vi "ex3.vi"() -> ()   [LabVIEW 2025]
panel:
  out "Numeric":i32
  in  "D":u32 format="%b"
  out "CRC 2":u32 format="%b"
  out "Message with CRC 2":u32 format="%b"
  out "Message":u32 format="%b"
  out "CRC":u32 format="%b"
  in  "Message with CRC":u32 format="%b"
  # "Decoder"
  # "Enkoder"
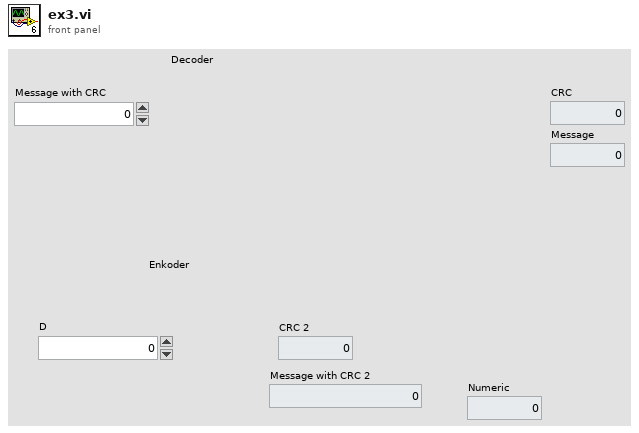
[diagram p1: front panel]
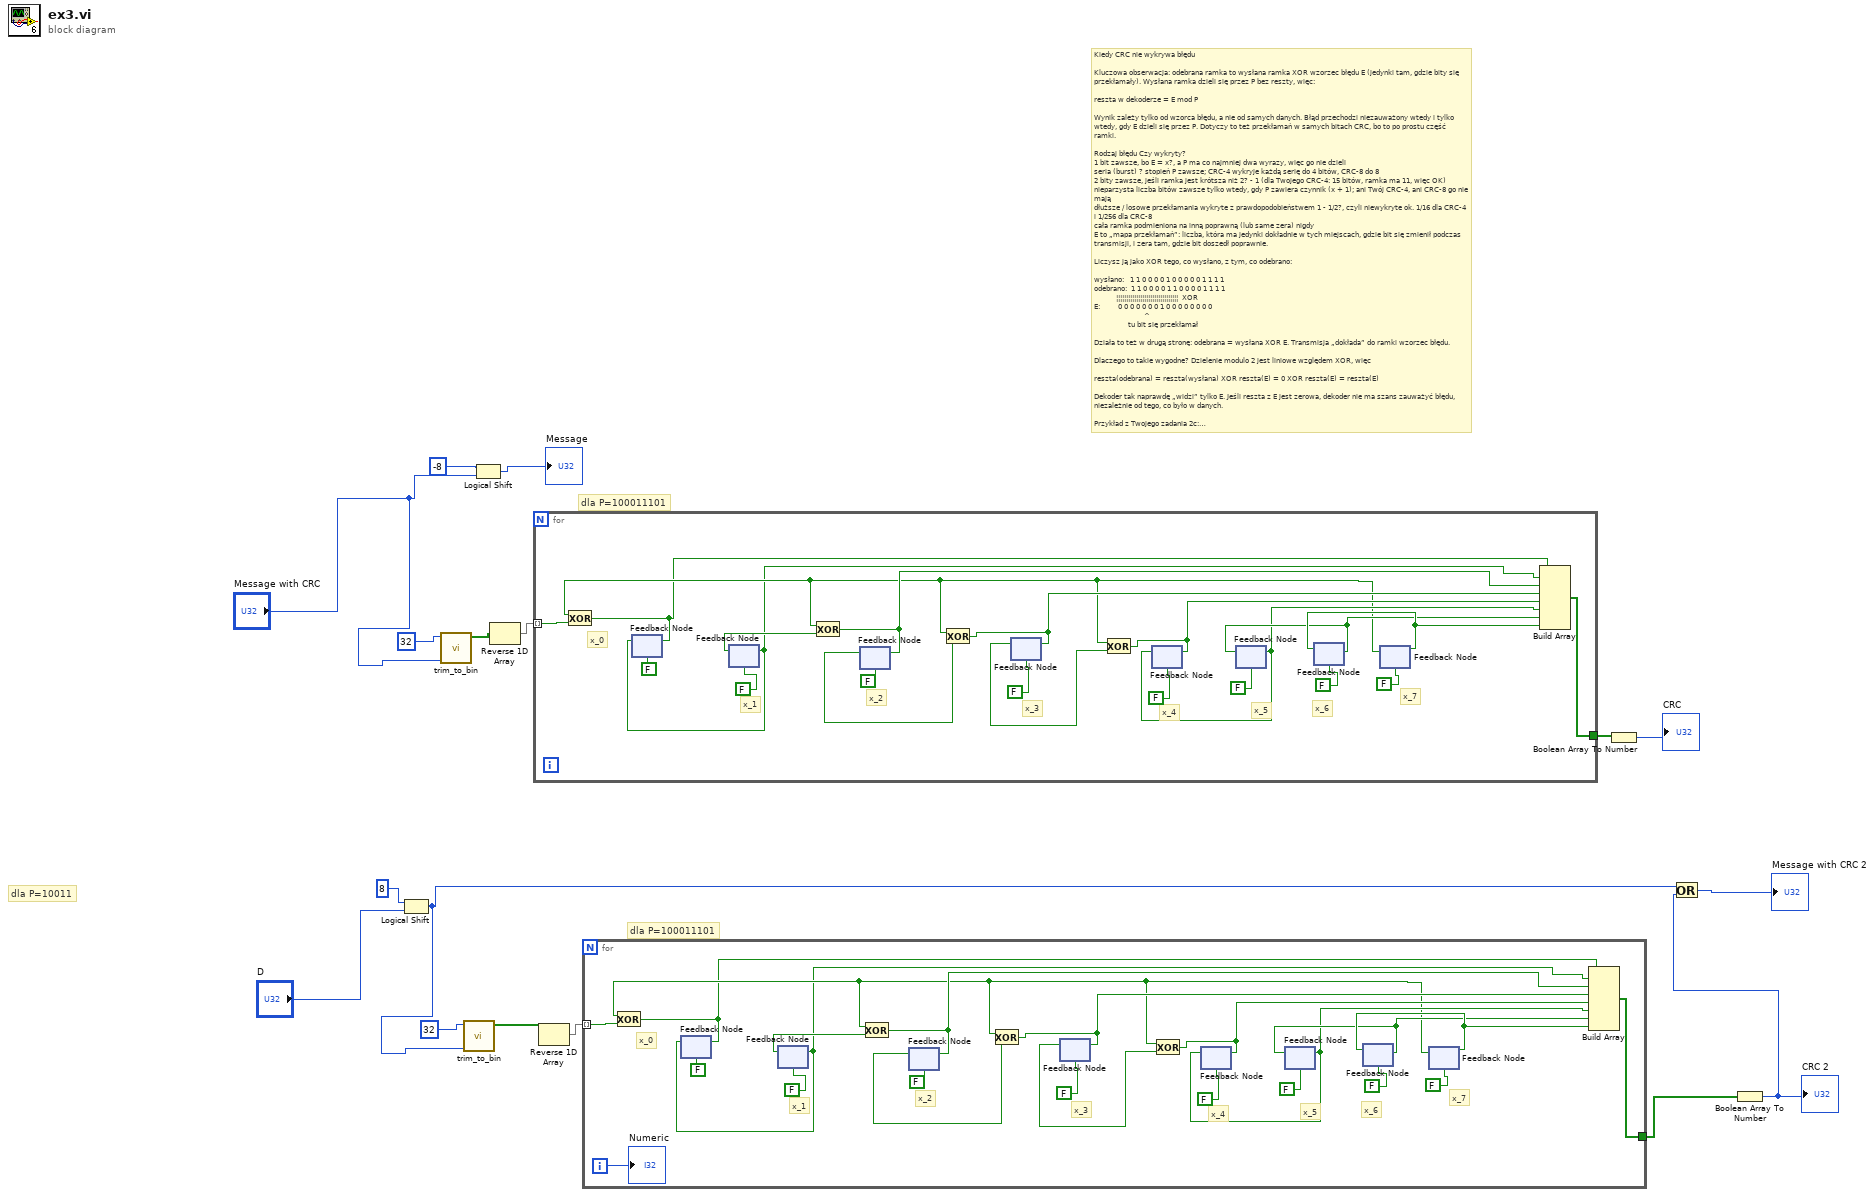
[diagram p0: block diagram]
diagram:
  # "Kiedy CRC nie wykrywa błędu\n\nKluczowa obserwacja: odebrana ramka to wysłana ramka XOR wzorzec błędu E (jedynki tam, gdzie bity się przekłamały). Wysłana ramka dzieli się przez P bez reszty, więc:\n\nreszta w dekoderze = E mod P\n\nWynik zależy tylko od wzorca błędu, a nie od samych danych. Błąd przechodzi niezauważony wtedy i tylko wtedy, gdy E dzieli się przez P. Dotyczy to też przekłamań w samych bitach CRC, bo to po prostu część ramki.\n\nRodzaj błędu\tCzy wykryty?\n1 bit\tzawsze, bo E = x?, a P ma co najmniej dwa wyrazy, więc go nie dzieli\nseria (burst) ? stopień P\tzawsze; CRC-4 wykryje każdą serię do 4 bitów, CRC-8 do 8\n2 bity\tzawsze, jeśli ramka jest krótsza niż 2? - 1 (dla Twojego CRC-4: 15 bitów, ramka ma 11, więc OK)\nnieparzysta liczba bitów\tzawsze tylko wtedy, gdy P zawiera czynnik (x + 1); ani Twój CRC-4, ani CRC-8 go nie mają\ndłuższe / losowe przekłamania\twykryte z prawdopodobieństwem 1 - 1/2?, czyli niewykryte ok. 1/16 dla CRC-4 i 1/256 dla CRC-8\ncała ramka podmieniona na inną poprawną (lub same zera)\tnigdy\nE to „mapa przekłamań”: liczba, która ma jedynki dokładnie w tych miejscach, gdzie bit się zmienił podczas transmisji, i zera tam, gdzie bit doszedł poprawnie.\n\nLiczysz ją jako XOR tego, co wysłano, z tym, co odebrano:\n\nwysłano:   1 1 0 0 0 0 1 0 0 0 0 0 1 1 1 1\nodebrano:  1 1 0 0 0 0 1 1 0 0 0 0 1 1 1 1\n           ¦¦¦¦¦¦¦¦¦¦¦¦¦¦¦¦¦¦¦¦¦¦¦¦¦¦¦¦¦¦¦  XOR\nE:         0 0 0 0 0 0 0 1 0 0 0 0 0 0 0 0\n                         ^\n                 tu bit się przekłamał\n\nDziała to też w drugą stronę: odebrana = wysłana XOR E. Transmisja „dokłada” do ramki wzorzec błędu.\n\nDlaczego to takie wygodne? Dzielenie modulo 2 jest liniowe względem XOR, więc\n\nreszta(odebrana) = reszta(wysłana) XOR reszta(E) = 0 XOR reszta(E) = reszta(E)\n\nDekoder tak naprawdę „widzi” tylko E. Jeśli reszta z E jest zerowa, dekoder nie ma szans zauważyć błędu, niezależnie od tego, co było w danych.\n\nPrzykład z Twojego zadania 2c:\n\nwysłano:   0 1 0 1 1 0 0 1 1 0 1 0   (10110011010 z zerem z przodu)\nodebrano:  1 0 0 1 1 1 0 0 1 1 0 0\nE:         1 1 0 0 0 1 0 1 0 1 1 0\n\nPrzekłamało się 6 bitów, ale ten wzorzec akurat dzieli się przez 10011, więc dekoder pokazał 0. Możesz to sprawdzić swoim enkoderem/dekoderem: podaj 110001010110 jako ramkę do dekodera i powinna wyjść reszta 0.\n\nPrzykład z Twojego laboratorium: błąd 3-bitowy o wzorcu dokładnie 10011 (= P) w dowolnym miejscu ramki CRC-4 przejdzie niezauważony, bo E = P·x?. Dla CRC-8 ten sam wzoriec zostanie już wykryty, bo 10011 nie dzieli się przez 100011101. Po to w zadaniu 3 jest „lepszy wielomian”: im wyższy stopień, tym mniej wzorców błędów jest podzielnych przez P."
  # "dla P=100011101"
  # "dla P=10011"
  # "dla P=100011101"
  n1 = Logical Shift(y=i16 8, x="D") -> (x << y=w4:u32)
  n2 = call "trim_to_bin.vi"("number"="Message with CRC", "constant"=u32 32) -> ("new array"=w16:bool[])  [unwired: 8 in, 1 out]
  n3 = call "trim_to_bin.vi"("number"=w4, "constant"=u32 32) -> ("new array"=w1:bool[])  [unwired: 8 in, 1 out]
  n4 = Logical Shift(y=i16 -8, x="Message with CRC") -> (x << y=→"Message":u32)
  n5 = Reverse 1D Array(array=w16) -> (reversed array=w15:bool[])
  n6 = for {
    tunnel: w15 -> [w39] mode=indexing
    tunnel: [w37] -> w14
    # "x_7"
    # "x_6"
    # "x_5"
    # "x_4"
    # "x_3"
    # "x_2"
    # "x_1"
    # "x_0"
    n7 = feedback #1(FALSE) -> (w19:bool)
    n8 = feedback #2(FALSE) -> (w35:bool)
    n9 = feedback-in #2(w19) -> ()
    n10 = feedback #3(FALSE) -> (w33:bool)
    n11 = feedback #4(FALSE) -> (w30:bool)
    n12 = feedback #5(FALSE) -> (w24:bool)
    n13 = feedback #6(FALSE) -> (w25:bool)
    n14 = feedback-in #6(w24) -> ()
    n15 = feedback #7(FALSE) -> (w26:bool)
    n16 = feedback-in #7(w25) -> ()
    n17 = feedback #8(FALSE) -> (w20:bool)
    n18 = Exclusive Or(1:w39, 2:w20) -> (0:w18:bool)
    n19 = feedback-in #1(w18) -> ()
    n20 = Exclusive Or(1:w35, 2:w20) -> (0:w21:bool)
    n21 = feedback-in #3(w21) -> ()
    n22 = Exclusive Or(1:w33, 2:w20) -> (0:w22:bool)
    n23 = feedback-in #4(w22) -> ()
    n24 = Exclusive Or(1:w30, 2:w20) -> (0:w23:bool)
    n25 = feedback-in #5(w23) -> ()
    n26 = feedback-in #8(w26) -> ()
    n27 = Build Array(w18, w19, w21, w22, w23, w24, w25, w26) -> (w37:bool[])
  }
  n28 = Reverse 1D Array(array=w1) -> (reversed array=w3:bool[])
  n29 = for {
    tunnel: w3 -> [w62] mode=indexing
    tunnel: [w60] -> w2
    i -> [w42]
    # "x_7"
    # "x_6"
    # "x_5"
    # "x_4"
    # "x_3"
    # "x_2"
    # "x_1"
    # "x_0"
    n30 = feedback #9(FALSE) -> (w41:bool)
    n31 = feedback #10(FALSE) -> (w58:bool)
    n32 = feedback-in #10(w41) -> ()
    n33 = feedback #11(FALSE) -> (w56:bool)
    n34 = feedback #12(FALSE) -> (w53:bool)
    n35 = feedback #13(FALSE) -> (w47:bool)
    n36 = feedback #14(FALSE) -> (w48:bool)
    n37 = feedback-in #14(w47) -> ()
    n38 = feedback #15(FALSE) -> (w49:bool)
    n39 = feedback-in #15(w48) -> ()
    n40 = feedback #16(FALSE) -> (w43:bool)
    n41 = Exclusive Or(1:w62, 2:w43) -> (0:w40:bool)
    n42 = feedback-in #9(w40) -> ()
    n43 = Exclusive Or(1:w58, 2:w43) -> (0:w44:bool)
    n44 = feedback-in #11(w44) -> ()
    n45 = Exclusive Or(1:w56, 2:w43) -> (0:w45:bool)
    n46 = feedback-in #12(w45) -> ()
    n47 = Exclusive Or(1:w53, 2:w43) -> (0:w46:bool)
    n48 = feedback-in #13(w46) -> ()
    n49 = feedback-in #16(w49) -> ()
    n50 = Build Array(w40, w41, w44, w45, w46, w47, w48, w49) -> (w60:bool[])
    "Numeric" <- w42
  }
  n51 = Boolean Array To Number(Boolean array=w14) -> (number=→"CRC":u32)
  n52 = Boolean Array To Number(Boolean array=w2) -> (number=w6:u32)
  "CRC 2" <- w6
  n53 = Or(x=w4, y=w6) -> (x .or. y?=→"Message with CRC 2":u32)
